vi "RemoteVI Server Loop.vi"(0 "VI":refnum<vi>, 1 "share":T7, 5 "port":u16=8088, 7 "fps":dbl=20.0, 9 "stop notifier name":string, 11 "error in":errorcluster) -> (15 "error out":errorcluster)   [LabVIEW 2020, in "RemoteVI.lvlib"]
doc: "The RemoteVI server: ONE While Loop, no event structure (docs\\architecture.md, tools\\mock-server\\server.mjs). REENTRANT (preallocated clone), so a LabVIEW application instance can run one per port. share.window not 0 makes it a WINDOW TARGET: that window of any process is shared instead of VI's front panel - over VI Server as the VI whose panel it is when its LabVIEW runs one (RemoteVI Server Setup.vi, status kind VI Server; modifier keys, tip strips and splitter bars then run inside that process through RemoteVI Remote Hooks.vi), else (Win32 only - capture, input, popups, other windows of its process, its geometry and whether it still exists; no tips, no splitters, no VI Server), so a LabVIEW application instance can run one per port. share holds the access token, the net address to listen on (127.0.0.1 for this computer only, 0 for the whole network), the link, view only and whole network. Before the loop it creates a TCP listener on port at share's net address and sends its error cluster on the notifier <stop notifier name>:started (RemoteVI Start.vi waits for it, so a port in use is reported to the caller), obtains the notifier named stop notifier name and builds the greeting from the name of VI (RemoteVI Greeting.vi). Each iteration: ACCEPT - waits at most 5 ms for a connection and hands it to RemoteVI Accept Clients.vi, which keeps accepted connections PENDING and reads their request heads with zero-timeout reads, serves a complete head (RemoteVI Handle Connection.vi, at most 8 WebSocket clients), greets and adds an upgraded connection as a client, and drops one that has sent no complete head within 5 s - so an idle connection (a browser's speculative preconnect) never stalls the loop. POPUPS (docs\\architecture.md, section Popups) - RemoteVI Track Popups.vi lists the LabVIEW popups (Win32 only - while a popup is open LabVIEW's UI thread is in a modal loop and every VI Server UI call blocks) whenever a client is connected, a popup was open last time or the geometry is due, hides on the host the popups a remote click opened (within 1 s) and tip strips that can only stem from the remote pointer, and gives the modal popups at their LOGICAL positions (real - d). WINDOWS (docs\\protocol.md section 7) - RemoteVI Track Windows.vi lists the application's other windows (dialogs, native file dialogs, subVI panels; Win32 only); while one of them is modal LabVIEW's UI thread runs the dialog's modal loop and the loop makes no VI Server call, exactly as while a popup is open. GEOMETRY - the panel geometry and window handle are cached (RemoteVI Get Panel Geometry.vi before the loop, then every 500 ms and right after a popup closes - RemoteVI Refresh Geometry.vi - but only while NO popup is open and not within 300 ms of a click). SERVICE - every client is serviced (RemoteVI Service Clients.vi) with the cached geometry, handle and popups; the displacement d it returns is kept for the next iteration (reset when the last popup closes). SECOND LISTING - after servicing and the hover, when a client posted a message that may open a popup or a popup is open, RemoteVI Retrack Popups.vi lists the popups once more, so a popup the input just opened is hidden on the host at once (layered with alpha 0, RemoteVI Hide Remote Popups.vi) and, when the popups changed, its OVERLAY goes out before this iteration's frame (RemoteVI Send Overlay.vi with period 0). HOVER - RemoteVI Menu Hover.vi applies the remote pointer a client moved over an open LabVIEW menu with keys (the highlight follows it with VK_DOWN / VK_UP, VK_RIGHT after 400 ms on an item opens its submenu, VK_LEFT closes submenus when the pointer rests on a parent) - no cursor and no menu is moved. SPLITTERS - LabVIEW moves a splitter bar only while it tracks the real mouse, so the browser drags the bars itself: right after each geometry refresh RemoteVI Read Splitters.vi reads the bars ({LV.Panel} Splitters[]) for the splitters message (a new client gets it with its greeting, all clients when it changed), and RemoteVI Apply Splitter.vi sets the Position of the bar a client dropped (s id pos, stored by RemoteVI Splitter Request.vi) whenever no popup and no modal window is open; after a move the bars and tips are read again and frames come every 16 ms. TIPS - right after each geometry refresh (so never while a popup or a modal window is open) RemoteVI Read Tips.vi reads the tip strips of the panel's controls through VI Server; a new client gets the tips message with its greeting and RemoteVI Send Tips.vi tells all clients when it changed (docs\\protocol.md 3.3). ORIGIN - where the panel starts inside the frame (below the menu bar and toolbar) is cached with the geometry; a new client gets it with its greeting (RemoteVI Origin Message.vi), and RemoteVI Send Origin.vi tells all clients when it changed. FRAMES - RemoteVI Capture And Send.vi makes a frame at most every 1000/fps ms while a client is connected - every 16 ms while a client posted a click or a key in this iteration or within the last 300 ms (recent click?), so the change it causes reaches the browser at once instead of up to one frame period later - and sends it to each client; a frame is the whole window below its title bar (menu bar, toolbar, panel, scrollbars), copied from the window's composited surface (RemoteVI Capture Frame.vi) - no VI Server call, so frames keep coming while a popup is open. OTHER WINDOWS - RemoteVI Send Windows.vi sends each client the list (windows [...]) when it changed and, in an iteration that made a frame, each window's changes as a WINDOW FRAME (seq and flow control shared with FRAME); input goes to the window RemoteVI Route Input.vi picks. OVERLAY - RemoteVI Send Overlay.vi sends the popups as an OVERLAY message when it changed (docs\\protocol.md section 3.2); not in an iteration that made a frame (its period is then 1e9 ms) but in the next one, 1 ms later - capturing and PNG-encoding the popups right after the frame made the iteration, and with it the frame gap, longer (measured). Closed clients are dropped and their connections closed (RemoteVI Drop Closed Clients.vi). While the panel window is disabled (a modal dialog is up, even before it is listed - a native file dialog takes a moment to appear) no VI Server call is made either, as such a call would wait for the dialog's modal loop; for a window of another LabVIEW over VI Server it would block the loop until the dialog closes. The loop stops when the notifier delivers anything, when VI is no longer running (RemoteVI VI Stopped.vi, once a second while VI Server may be called - so the server ends with your application), or on a listener error other than a timeout. Then every client gets close 1001, every connection and the listener are closed and the notifier released, and the share's entry is removed from the status (RemoteVI Publish Status.vi, which publishes it every 500 ms while the loop runs). Launched asynchronously by RemoteVI Start.vi."
uses:
  RemoteVI.lvlib
panel:
  in  "windows not listed yet":T1
  in  "no windows":T2(array[cluster])
  in  "no popup windows":u64[](array[numeric])
  in  "no bars":T3(array[cluster])
  in  "no capture yet":T4
  in  "nothing pending":T5(array[cluster])
  in  "no clients":T6(array[cluster])
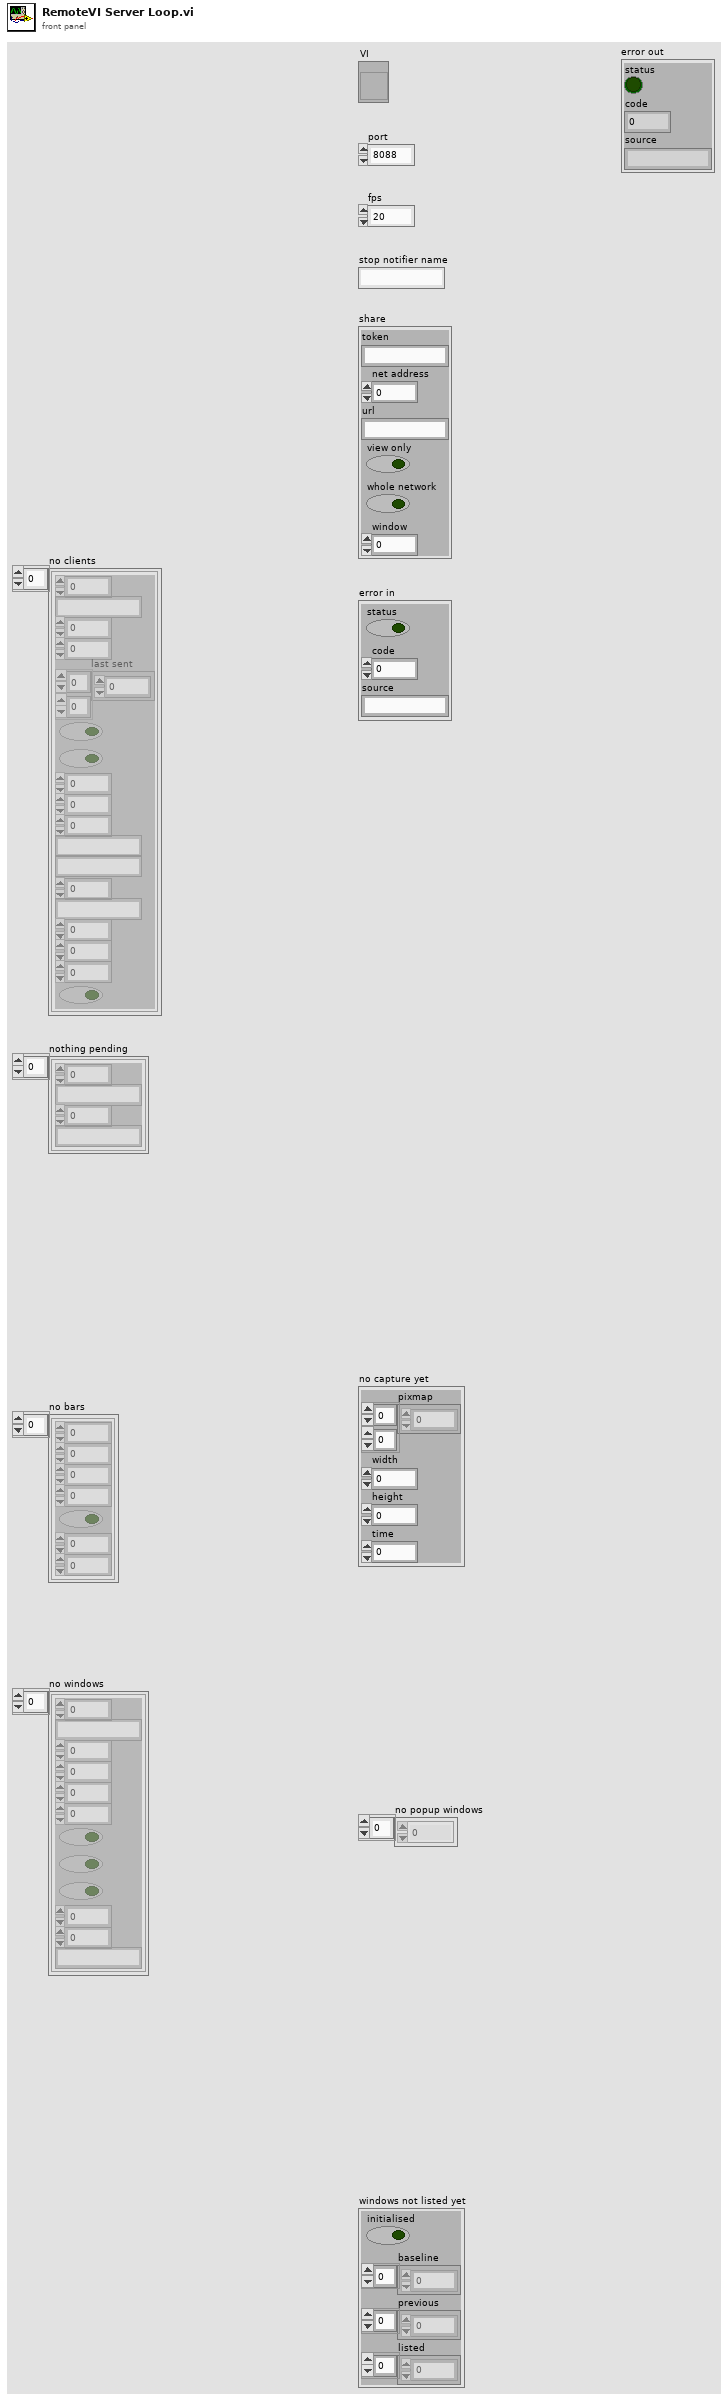
[diagram p1: front panel]
types:
  T1 = cluster{"initialised":bool, "baseline":u64[], "previous":u64[], "listed":u64[]}
  T2 = cluster{"id":u64, "title":string, "x":i32, "y":i32, "w":i32, "h":i32, "modal":bool, "active":bool, "closable":bool, "sx":i32, "sy":i32, "class":string}[]
  T3 = cluster{"x":i32, "y":i32, "w":i32, "h":i32, "vertical":bool, "min":i32, "max":i32}[]
  T4 = cluster{"pixmap":u32[][], "width":i32, "height":i32, "time":u32}
  T5 = cluster{"connection":u32, "head":string, "accepted":u32, "address":string}[]
  T6 = cluster{"connection":u32, "rx buffer":string, "seq":u32, "acked":u32, "last sent":u32[][], "tracking":bool, "closed":bool, "mods":u8, "mods set":u8, "popup since":u32, "windows sent":string, "window frames":cluster{"id":u64, "pixels":u32[][]}[], "key window":u64, "address":string, "since":dbl, "last input":dbl, "bytes":dbl, "view only":bool}[]
  T7 = cluster{"token":string, "net address":u32, "url":string, "view only":bool, "whole network":bool, "window":u64}
  T8 = cluster{"message":string, "frame":string, "time":u32}
  T9 = cluster{"last":dbl, "frames":u32, "frames last":u32, "bytes last":dbl, "click at":dbl, "latency":dbl, "fps":dbl, "rate":dbl}
  T10 = cluster{"port":u16, "url":string, "target":string, "kind":string, "whole network":bool, "view only":bool}
  T11 = cluster{"panelX":i32, "panelY":i32, "clientX":i32, "clientY":i32}
  T12 = cluster{"windows":cluster{"hwnd":u64, "x":i32, "y":i32, "w":i32, "h":i32}[], "dx":i32, "dy":i32}
  T13 = cluster{"hwnd":u64, "x":i32, "y":i32, "w":i32, "h":i32, "class":string}[]
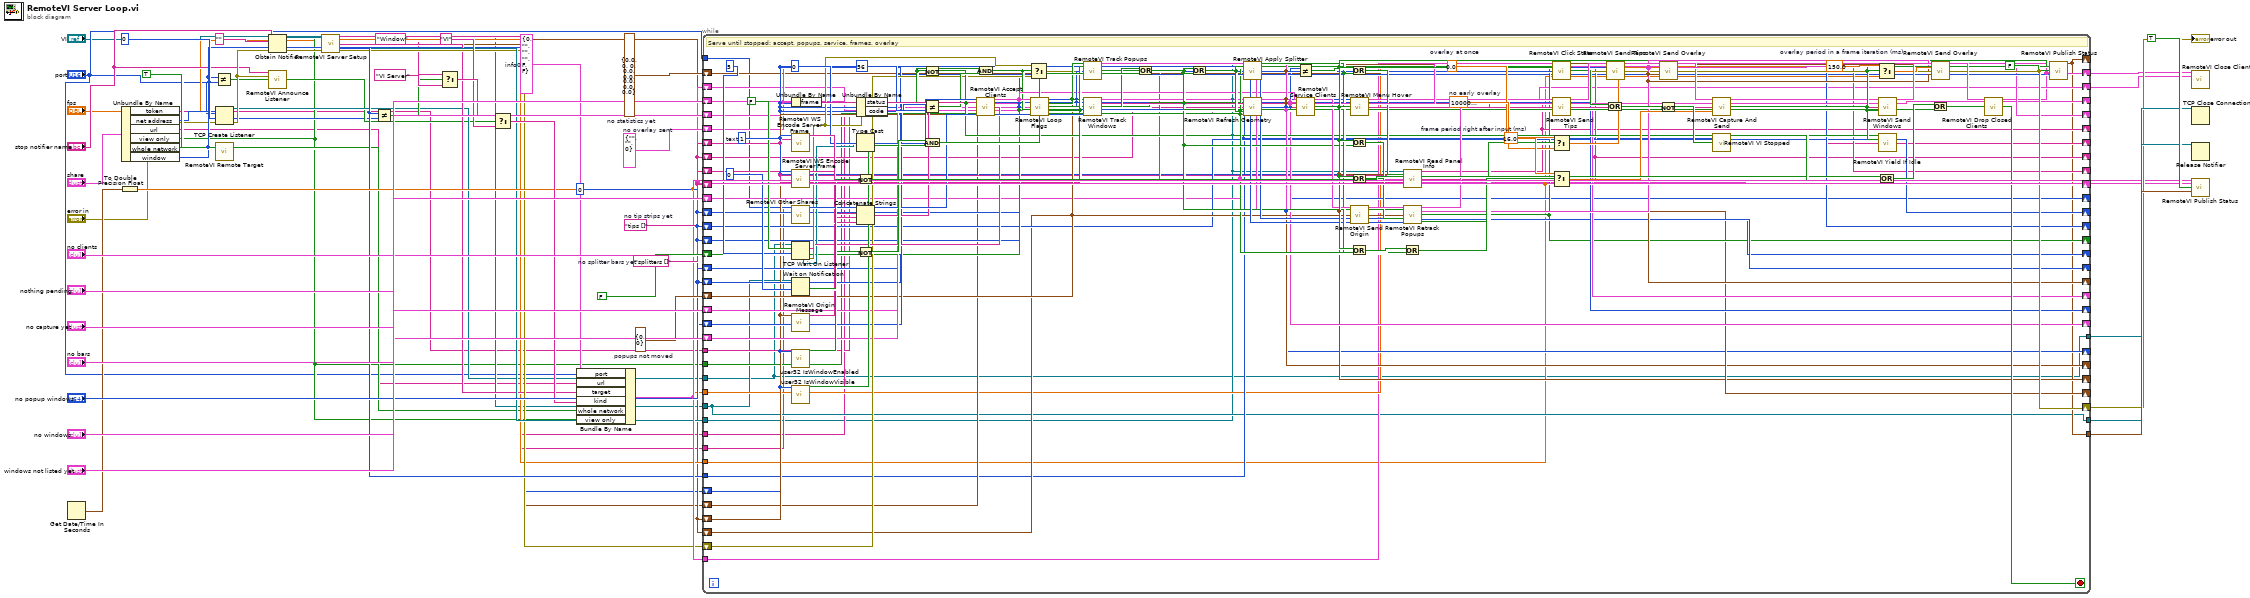
[diagram p0: block diagram]
diagram:
  w51 = cluster{"dx":i32, "dy":i32} {"dx"=0, "dy"=0}  # popups not moved
  w47 = "splitters []"  # no splitter bars yet
  w46 = "tips []"  # no tip strips yet
  w45 = u32 0
  w44 = T8 {"message"="", "frame"="", "time"=0}  # no overlay sent
  w40 = T9 {"last"=0.0, "frames"=0, "frames last"=0, "bytes last"=0.0, "click at"=0.0, "latency"=0.0, "fps"=0.0, "rate"=0.0}  # no statistics yet
  w38 = T10 {"port"=0, "url"="", "target"="", "kind"="", "whole network"=FALSE, "view only"=FALSE}  # info0
  w13 = u64 0
  n1 = Get Date/Time In Seconds() -> (seconds since 1Jan1904=w31:timestamp)
  n2 = Unbundle By Name("share") -> ("token"=w7:string, "net address"=w8:u32, "url"=w9:string, "view only"=w10:bool, "whole network"=w11:bool, "window"=w12:u64)
  n3 = To Double Precision Float(number=w31) -> (double precision float=w32:dbl)
  n4 = Not Equal?(x=w12, y=w13) -> (x != y?=w14:bool)
  n5 = TCP Create Listener(7:w8, 8:"error in", 10:"port") -> (0:w17:errorcluster, 3:w16:refnum<k5>)  [unwired: 2 in, 1 out]
  n6 = call "RemoteVI Remote Target.vi"("hWnd"=w12, "remove?"=TRUE) -> ()  [unwired: 11 in, 3 out]
  n7 = Obtain Notifier(name (unnamed)="stop notifier name", notification data type="", error in (no error)=w17) -> (notifier out=w19:refnum<notifier>, error out=w20:errorcluster)  [unwired: 1 in, 1 out]
  n8 = call "RemoteVI Announce Listener.vi"("stop notifier name"="stop notifier name", "listener result"=w17) -> ()  [unwired: 14 in]
  n9 = call "RemoteVI Server Setup.vi"("VI"="VI", "view only?"=w10, "fps"="fps", "window"=w12, "error in"=w20) -> ("origin"=w25:cluster{"x":i32, "y":i32}, "period"=w26:dbl, "hello"=w21:string, "html"=w22:string, "VI name"=w27:string, "geo"=w23:T11, "hWnd"=w24:u64, "VI out"=w29:refnum<vi>, "window out"=w30:u64, "error out"=w28:errorcluster)  [unwired: 1 out]
  n10 = Not Equal?(x=w30, y=w13) -> (x != y?=w34:bool)
  n11 = Select(t="Window", s=w34, f="VI Server") -> (s? t:f=w36:string)
  n12 = Select(t=w36, s=w14, f="VI") -> (s? t:f=w37:string)
  n13 = Bundle By Name(cluster=w38, "port"="port", "url"=w9, "target"=w27, "kind"=w37, "whole network"=w11, "view only"=w10) -> (w39:T10)
  n14 = while {
    tunnel: "port" -> [w72]
    shift-right: [w75] -> _
    shift-left: w40 -> [w74]
    shift-right: [w77] -> w54
    shift-left: "no clients" -> [w76]
    shift-right: [w79] -> w55
    shift-left: "nothing pending" -> [w78]
    shift-right: [w81] -> _
    shift-left: "no capture yet" -> [w80]
    shift-right: [w83] -> _
    shift-left: w44 -> [w82]
    shift-right: [w91] -> _
    shift-left: w46 -> [w90]
    shift-right: [w93] -> _
    shift-left: w46 -> [w92]
    shift-right: [w95] -> _
    shift-left: w47 -> [w94]
    shift-right: [w97] -> _
    shift-left: w47 -> [w96]
    shift-right: [w99] -> _
    shift-left: "no bars" -> [w98]
    shift-right: [w103] -> _
    shift-left: w45 -> [w102]
    shift-right: [w105] -> _
    shift-left: w45 -> [w104]
    shift-right: [w107] -> _
    shift-left: w45 -> [w106]
    shift-right: [w109] -> _
    shift-left: FALSE -> [w108]
    shift-right: [w111] -> _
    shift-left: "no popup windows" -> [w110]
    shift-right: [w113] -> _
    shift-left: "no popup windows" -> [w112]
    shift-right: [w115] -> _
    shift-left: w51 -> [w114]
    shift-right: [w117] -> _
    shift-left: "windows not listed yet" -> [w116]
    shift-right: [w119] -> _
    shift-left: w45 -> [w118]
    shift-right: [w121] -> _
    shift-left: "no windows" -> [w120]
    tunnel: w7 -> [w68]
    tunnel: w10 -> [w69]
    tunnel: w16 -> [w62]
    tunnel: w32 -> [w71]
    tunnel: w19 -> [w67]
    tunnel: [w62] -> w57
    tunnel: w29 -> [w63]
    tunnel: w22 -> [w64]
    tunnel: w21 -> [w65]
    tunnel: w26 -> [w66]
    tunnel: w30 -> [w73]
    shift-right: [w85] -> _
    shift-left: w24 -> [w84]
    shift-right: [w87] -> _
    shift-left: w23 -> [w86]
    shift-right: [w89] -> _
    shift-left: w25 -> [w88]
    shift-right: [w101] -> _
    shift-left: w25 -> [w100]
    shift-right: [w123] -> w56
    shift-left: w28 -> [w122]
    tunnel: [w67] -> w58
    tunnel: w39 -> [w70]
    tunnel: [w75] -> w59
    stop <- w200 stop-if-true
    w188 = 150.0  # overlay period in a frame iteration (ms)
    w182 = 16.0  # frame period right after input (ms)
    w178 = 1000000000.0  # no early overlay
    w177 = 0.0  # overlay at once
    w139 = u8 1  # text
    # "Serve until stopped: accept, popups, service, frames, overlay"
    n15 = Unbundle By Name(w82) -> ("frame"=w137:string)
    n16 = call "RemoteVI WS Encode Server Frame.vi"("opcode"=w139, "payload"=w90) -> ("frame"=w140:string)  [unwired: 13 in]
    n17 = call "RemoteVI WS Encode Server Frame.vi"("opcode"=w139, "payload"=w94) -> ("frame"=w141:string)  [unwired: 13 in]
    n18 = call "RemoteVI Other Shares.vi"("port"=w72) -> ("hWnds"=w154:u64[])  [unwired: 14 in]
    n19 = TCP Wait On Listener(9:5, 10:FALSE, 11:w62) -> (0:w128:errorcluster, 2:w127:string, 4:w126:refnum<k5>)  [unwired: 1 in, 2 out]
    n20 = Wait on Notification(notifier=w67, timeout in ms (-1)=0) -> (timed out?=w194:bool)  [unwired: 2 in, 3 out]
    n21 = call "RemoteVI Origin Message.vi"("origin"=w88) -> ("frame"=w138:string)  [unwired: 14 in]
    n22 = call "user32 IsWindowEnabled.vi"("hWnd"=w84) -> ("enabled?"=w157:bool)  [unwired: 13 in, 1 out]
    n23 = call "user32 IsWindowVisible.vi"("hWnd"=w84) -> ("visible?"=w158:bool)  [unwired: 13 in, 1 out]
    n24 = Unbundle By Name(w128) -> ("status"=w129:bool, "code"=w130:i32)
    n25 = Type Cast(type=u32 0, x=w126) -> (*(type *) &x=w136:u32)
    n26 = Not(x=w194) -> (.not. x?=w195:bool)
    n27 = Concatenate Strings(w65, w138, w140, w141) -> (w142:string)
    n28 = Not(x=w157) -> (.not. x?=w159:bool)
    n29 = Not(x=w129) -> (.not. x?=w131:bool)
    n30 = Not Equal?(x=w130, y=56) -> (x != y?=w133:bool)
    n31 = And(x=w159, y=w158) -> (x .and. y?=w160:bool)
    n32 = And(x=w129, y=w133) -> (x .and. y?=w134:bool)
    n33 = call "RemoteVI Accept Clients.vi"("new connection"=w136, "html"=w64, "hello"=w142, "overlay frame"=w137, "accepted?"=w131, "pending"=w78, "new address"=w127, "clients"=w76, "token"=w68, "view only?"=w69, "hWnd"=w84) -> ("pending out"=w79:T5, "clients out"=w143:T6)  [unwired: 3 in]
    n34 = Select(t=w128, s=w134, f=w122) -> (s? t:f=w123:errorcluster)
    n35 = call "RemoteVI Loop Flags.vi"("clients"=w143, "last geometry"=w102, "last click"=w106, "popup was open?"=w108) -> ("now"=w144:u32, "look?"=w145:bool, "geometry due?"=w146:bool, "remote click?"=w147:bool, "recent click?"=w148:bool)  [unwired: 7 in]
    n36 = call "RemoteVI Track Popups.vi"("look?"=w145, "previously hidden"=w112, "remote click?"=w147, "panel hWnd"=w84, "d"=w114, "previous popup hWnds"=w110) -> ("hidden hWnds"=w153:u64[], "popups"=w149:T12, "overlay popups"=w150:T13, "popup open?"=w151:bool, "popup hWnds"=w152:u64[])  [unwired: 5 in]
    n37 = call "RemoteVI Track Windows.vi"("look?"=w145, "now"=w144, "last list"=w118, "panel hWnd"=w84, "state"=w116, "previous windows"=w120, "other shares"=w154) -> ("last list out"=w119:u32, "windows"=w121:T2, "message"=w155:string, "modal?"=w156:bool, "state out"=w117:T1)  [unwired: 4 in]
    n38 = Or(x=w156, y=w160) -> (x .or. y?=w161:bool)
    n39 = Or(x=w151, y=w161) -> (x .or. y?=w162:bool)
    n40 = call "RemoteVI Apply Splitter.vi"("VI"=w63, "hWnd"=w84, "bars"=w98, "busy?"=w162) -> ("moved?"=w163:bool)  [unwired: 11 in]
    n41 = call "RemoteVI Refresh Geometry.vi"("VI"=w63, "now"=w144, "geometry due?"=w146, "popup was open?"=w108, "geo"=w86, "hWnd"=w84, "last refresh"=w102, "origin"=w88, "popup open?"=w162, "recent click?"=w148, "window"=w73) -> ("geo out"=w87:T11, "hWnd out"=w85:u64, "last refresh out"=w103:u32, "origin out"=w89:cluster{"x":i32, "y":i32})  [unwired: 1 in]
    n42 = Not Equal?(x=w103, y=w102) -> (x != y?=w164:bool)
    n43 = call "RemoteVI Service Clients.vi"("clients"=w143, "windows"=w121, "geo"=w87, "hWnd"=w85, "popups"=w149) -> ("clients out"=w166:T6, "popups out"=w167:T12, "clicked?"=w168:bool)  [unwired: 8 in]
    n44 = Or(x=w164, y=w163) -> (x .or. y?=w165:bool)
    n45 = call "RemoteVI Menu Hover.vi"("hWnd"=w85, "popup open?"=w151, "clicked?"=w168) -> ()  [unwired: 13 in]
    n46 = Or(x=w168, y=w151) -> (x .or. y?=w169:bool)
    n47 = Or(x=w168, y=w147) -> (x .or. y?=w170:bool)
    n48 = call "RemoteVI Send Origin.vi"("clients"=w166, "origin"=w89, "origin sent"=w100) -> ("clients out"=w174:T6, "origin sent out"=w101:cluster{"x":i32, "y":i32})  [unwired: 11 in]
    n49 = Or(x=w168, y=w148) -> (x .or. y?=w183:bool)
    n50 = call "RemoteVI Read Panel Info.vi"("VI"=w63, "hWnd"=w84, "refresh?"=w165, "origin"=w89, "tips in"=w90, "splitters in"=w94, "bars in"=w98) -> ("tips out"=w91:string, "splitters out"=w95:string, "bars out"=w99:T3)  [unwired: 6 in]
    n51 = call "RemoteVI Retrack Popups.vi"("again?"=w169, "popups"=w149, "overlay popups"=w150, "popup open?"=w151, "panel hWnd"=w85, "d"=w114, "remote click?"=w170, "popup hWnds"=w152, "hidden hWnds"=w153) -> ("overlay popups out"=w171:T13, "popup open? out"=w109:bool, "popup hWnds out"=w111:u64[], "hidden hWnds out"=w113:u64[], "changed?"=w172:bool)  [unwired: 1 in, 1 out]
    n52 = Or(x=w183, y=w163) -> (x .or. y?=w184:bool)
    n53 = call "RemoteVI Click State.vi"("popups out"=w167, "recent click?"=w148, "popup open?"=w109, "clicked?"=w168, "now"=w144, "last click"=w106) -> ("d"=w115:cluster{"dx":i32, "dy":i32}, "last click out"=w107:u32, "no VI Server?"=w173:bool)  [unwired: 7 in]
    n54 = call "RemoteVI Send Tips.vi"("clients"=w174, "message"=w91, "message sent"=w92) -> ("clients out"=w175:T6, "message sent out"=w93:string)  [unwired: 11 in]
    n55 = Select(t=w177, s=w172, f=w178) -> (s? t:f=w179:dbl)
    n56 = Select(t=w182, s=w184, f=w66) -> (s? t:f=w185:dbl)
    n57 = call "RemoteVI Send Tips.vi"("clients"=w175, "message"=w95, "message sent"=w96) -> ("clients out"=w176:T6, "message sent out"=w97:string)  [unwired: 11 in]
    n58 = Or(x=w173, y=w161) -> (x .or. y?=w196:bool)
    n59 = call "RemoteVI Send Overlay.vi"("clients"=w176, "state"=w82, "period"=w179, "overlay popups"=w171, "geo"=w87, "d"=w115) -> ("clients out"=w180:T6, "state out"=w181:T8)  [unwired: 8 in]
    n60 = Not(x=w196) -> (.not. x?=w197:bool)
    n61 = call "RemoteVI Capture And Send.vi"("clients"=w180, "hWnd"=w85, "cache"=w80, "period"=w185) -> ("clients out"=w186:T6, "cache out"=w81:T4, "captured?"=w187:bool)  [unwired: 9 in]
    n62 = call "RemoteVI VI Stopped.vi"("VI"=w63, "window"=w73, "last check"=w104, "VI Server ok?"=w197) -> ("stopped?"=w198:bool, "last check out"=w105:u32)  [unwired: 10 in]
    n63 = Select(t=w188, s=w187, f=w66) -> (s? t:f=w189:dbl)
    n64 = call "RemoteVI Send Windows.vi"("clients"=w186, "windows"=w121, "message"=w155, "capture?"=w187) -> ("clients out"=w190:T6)  [unwired: 11 in]
    n65 = call "RemoteVI Yield If Idle.vi"("accepted?"=w131, "captured?"=w187) -> ()  [unwired: 14 in]
    n66 = Or(x=w195, y=w198) -> (x .or. y?=w199:bool)
    n67 = call "RemoteVI Send Overlay.vi"("clients"=w190, "state"=w181, "period"=w189, "overlay popups"=w171, "geo"=w87, "d"=w115) -> ("clients out"=w191:T6, "state out"=w83:T8)  [unwired: 8 in]
    n68 = Or(x=w199, y=w134) -> (x .or. y?=w200:bool)
    n69 = call "RemoteVI Drop Closed Clients.vi"("clients"=w191) -> ("clients out"=w77:T6)  [unwired: 14 in]
    n70 = call "RemoteVI Publish Status.vi"("info"=w70, "started"=w71, "clients"=w77, "captured?"=w187, "clicked?"=w168, "error"=w123, "stop?"=FALSE, "state"=w74, "hWnd"=w85) -> ("state out"=w75:T9)  [unwired: 6 in]
  }
  "error out" <- w56
  n71 = call "RemoteVI Close Clients.vi"("clients"=w54, "pending"=w55) -> ()  [unwired: 14 in]
  n72 = TCP Close Connection(connection ID=w57) -> ()  [unwired: 2 in, 2 out]
  n73 = Release Notifier(notifier=w58) -> ()  [unwired: 2 in, 3 out]
  n74 = call "RemoteVI Publish Status.vi"("info"=w39, "started"=w32, "clients"="no clients", "stop?"=TRUE, "state"=w59) -> ()  [unwired: 10 in, 1 out]
